vi "Analyze Dummy Module.vi"(8 "error in":errorcluster) -> (0 "error out":errorcluster, 3 "Analysis Output":T1)   [LabVIEW 2026]
doc: "This is a helper VI that analyzes the dummy module of the project and returns type definitions and functions."
uses:
  Type Definitions/Analysis Output--cluster.ctl
  Type Definitions/Type Definition--cluster.ctl
  Type Definitions/Parameter--cluster.ctl
  Type Definitions/Function--cluster.ctl
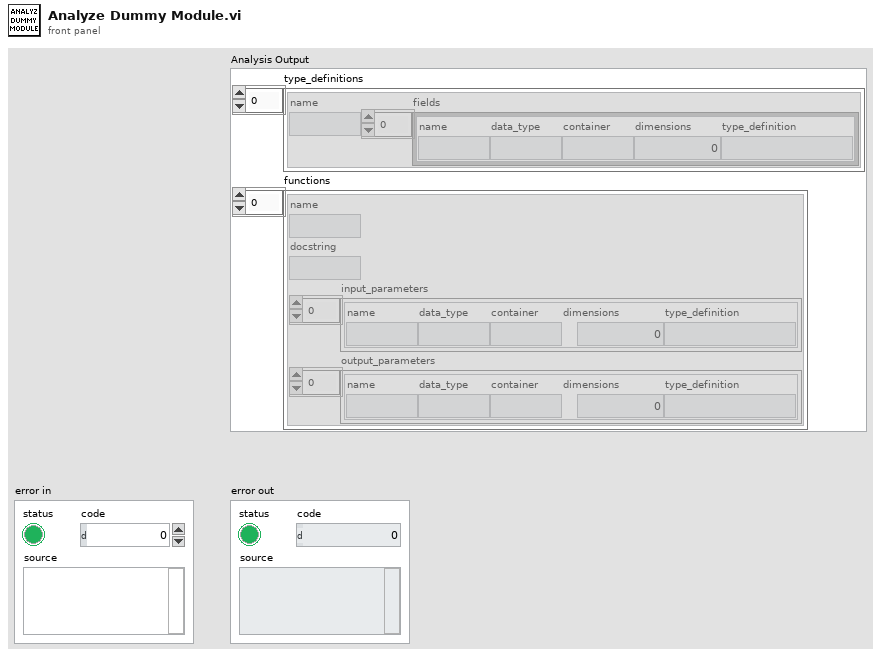
[diagram p1: front panel]
types:
  T1 = typedef "Analysis Output--cluster.ctl" = cluster{"type_definitions":T2[], "functions":T4[]}
  T2 = typedef "Type Definition--cluster.ctl" = cluster{"name":string, "fields":T3[]}
  T3 = typedef "Parameter--cluster.ctl" = cluster{"name":string, "data_type":string, "container":string, "dimensions":i32, "type_definition":string}
  T4 = typedef "Function--cluster.ctl" = cluster{"name":string, "docstring":string, "input_parameters":T3[], "output_parameters":T3[]}
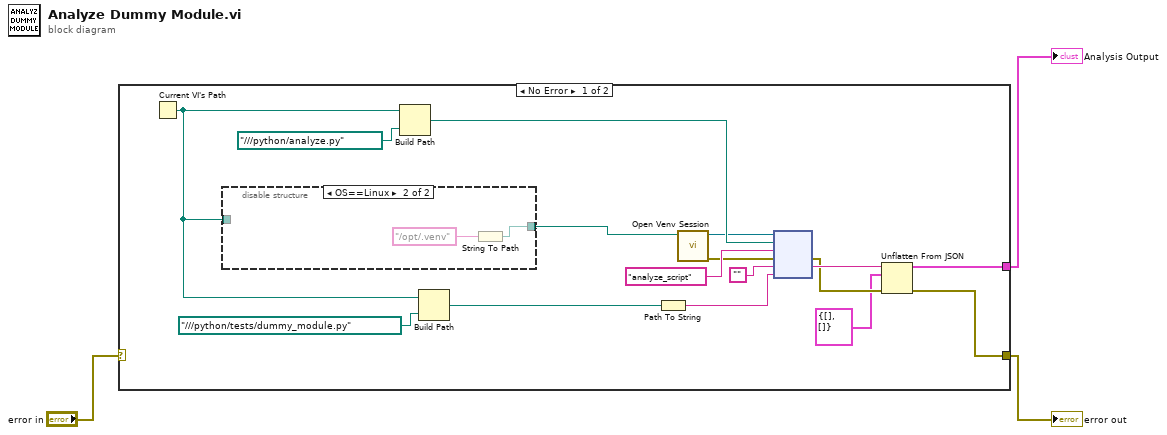
[diagram p0: block diagram]
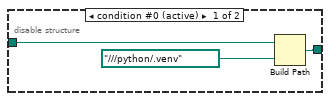
[diagram p2: hidden frame]
diagram:
  n1 = case shown="No Error" "error in" {
    selector: "error in" -> [_ w25]
    tunnel: [w7 _] -> w3
    tunnel: [w6 w25] -> w1
    frame No Error {
      n2 = Current VI's Path() -> (path=w5:path)
      n3 = disable-structure shown="OS==Linux" {
        disable-tunnel: w5 -> [w21 _]
        disable-tunnel: [w20 w23] -> w4
        frame condition #0 (active) {
          n4 = Build Path(base path=w21, name or relative path=path "../../../python/.venv") -> (appended path=w20:path)
        }
        frame condition #1 {
          n5 = String To Path(string="/opt/.venv") -> (path=w23:path)
        }
      }
      n6 = Build Path(base path=w5, name or relative path=path "../../../python/analyze.py") -> (appended path=w18:path)
      n7 = Build Path(base path=w5, name or relative path=path "../../../python/tests/dummy_module.py") -> (appended path=w14:path)
      n8 = Path To String(path=w14) -> (string=w13:string)
      n9 = call "Open Venv Session.vi"("Venv"=w4) -> ("error out"=w8:errorcluster, "session out"=w9:refnum<k35>)  [unwired: 9 in]
      n10 = node ("Python Node")(w9, w18, "analyze_script" ("function name"), w8, "" ("Empty String Constant"), w13) -> (w11:errorcluster, w12:string)  [unwired: 1 in, 3 out]
      n11 = Unflatten From JSON(JSON string=w12, type and defaults=T1 {"type_definitions"=[], "functions"=[]} ("Analysis Output"), error in (no error)=w11) -> (value=w7:T1, error out=w6:errorcluster)  [unwired: 4 in]
    }
    frame Error {
      # "Pass error without further action."
    }
  }
  "Analysis Output" <- w3
  "error out" <- w1
